vi "fake tool annotated.vi"(11 "value":string) -> (3 "echo":string)   [LabVIEW 2020, in "MCP Server tests.lvlib"]
doc: "Fake tool to test the title and the annotations of a tool. It is registered with a title and with readOnlyHint true and destructiveHint false; it only echoes its input."
uses:
  MCP Server tests.lvlib
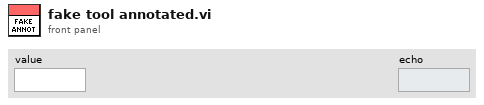
[diagram p1: front panel]
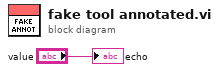
[diagram p0: block diagram]
diagram:
  "echo" <- "value"
